vi "traffic light using flat sequence.vi"() -> ()   [LabVIEW 2018]
panel:
  in  "stop":bool
  out "Green":bool
  out "Yellow":bool
  out "Red":bool
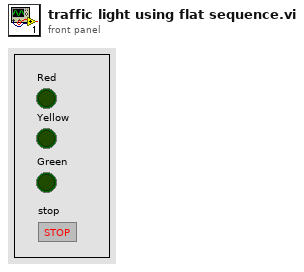
[diagram p1: front panel]
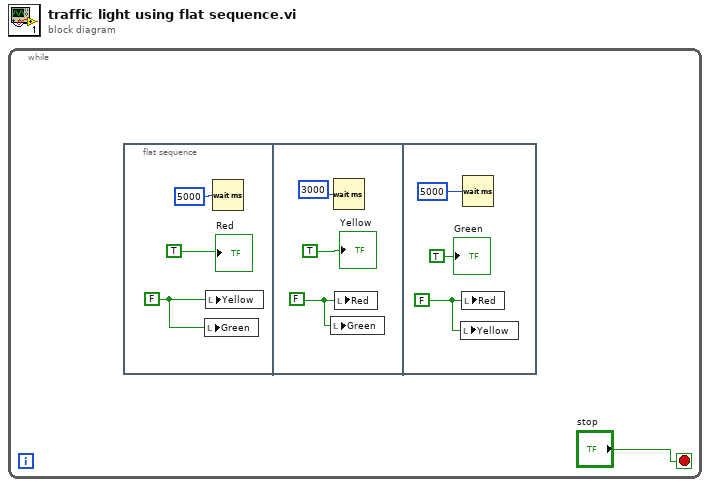
[diagram p0: block diagram]
diagram:
  n1 = while {
    stop <- "stop" stop-if-true
    n2 = flat-sequence {
      frame #0 {
        w2 = FALSE
        n3 = local write "Green"(w2) -> ()
        n4 = local write "Yellow"(w2) -> ()
        n5 = Wait (ms)(milliseconds to wait=5000) -> ()  [unwired: 1 out]
        "Red" <- TRUE ("Red")
      }
      frame #1 {
        w5 = FALSE
        n6 = local write "Green"(w5) -> ()
        n7 = Wait (ms)(milliseconds to wait=3000) -> ()  [unwired: 1 out]
        n8 = local write "Red"(w5) -> ()
        "Yellow" <- TRUE ("Yellow")
      }
      frame #2 {
        w8 = FALSE
        n9 = local write "Yellow"(w8) -> ()
        n10 = local write "Red"(w8) -> ()
        n11 = Wait (ms)(milliseconds to wait=5000) -> ()  [unwired: 1 out]
        "Green" <- TRUE ("Green")
      }
    }
  }
